vi "Create Indicator in Result.vi"(0 "Result Cluster":refnum<vi>, 1 "Output Clusters in":string[](array[string]), 5 "VI Reference":refnum<vi>, 7 "Ctl Refnum":refnum<vi>, 11 "error in (no error)":errorcluster) -> (4 "Output Clusters out":string[](array[string]), 15 "error out":errorcluster)   [LabVIEW 2021, in "Migrator.lvlib"]
uses:
  Migrator.lvlib
  <vilib>/Utility/miscctls.llb/LVPositionTypeDef.ctl
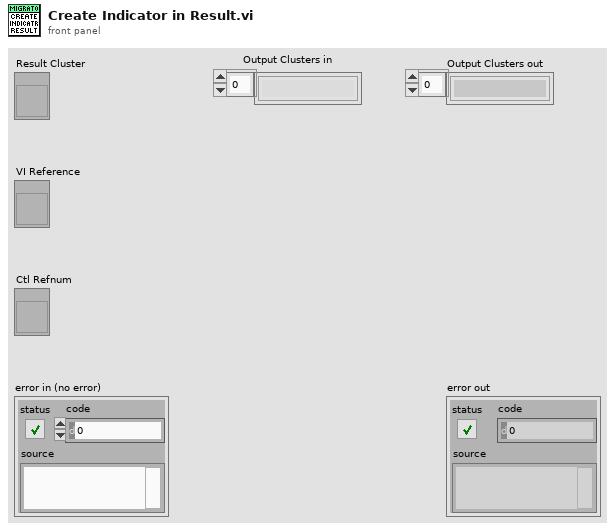
[diagram p1: front panel]
types:
  T1 = typedef "LVPositionTypeDef.ctl" = cluster{"Left":i32, "Top":i32}
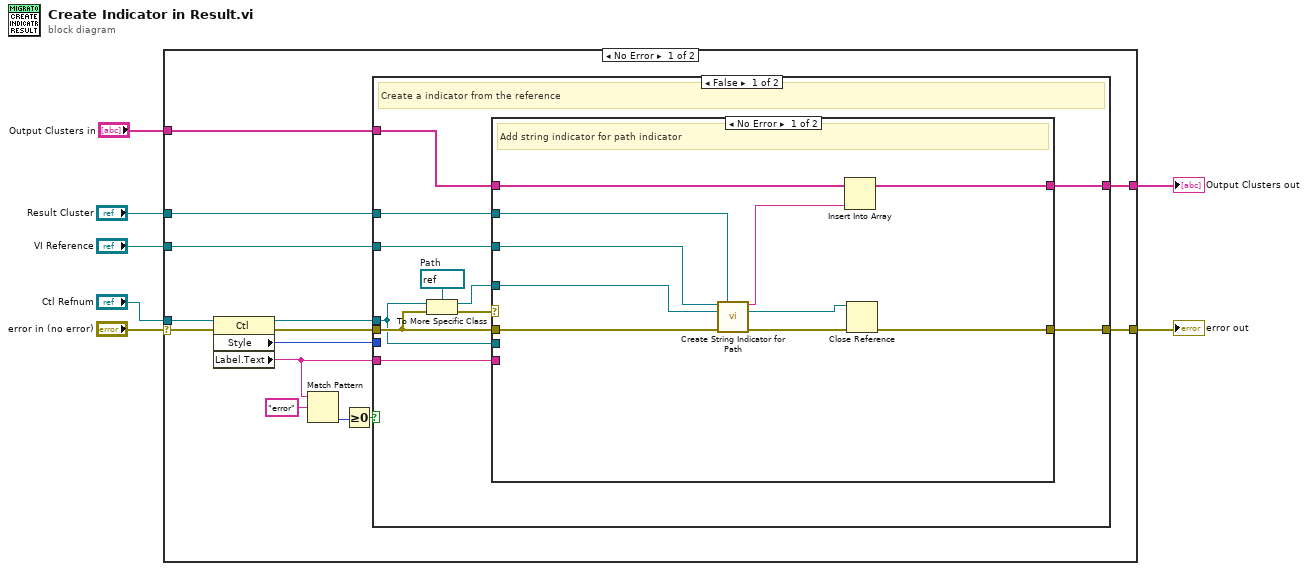
[diagram p0: block diagram]
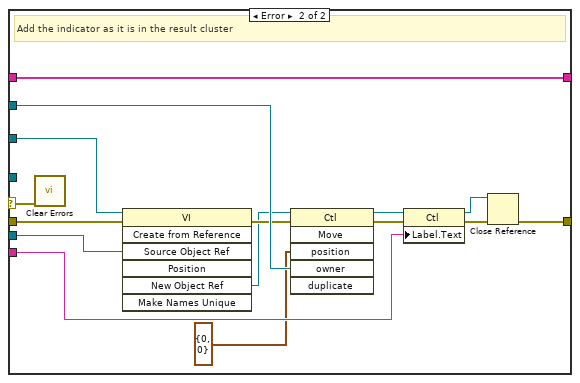
[diagram p2: hidden frame]
diagram:
  n1 = case shown="No Error" "error in (no error)" {
    selector: "error in (no error)" -> [w21 w61]
    tunnel: "Ctl Refnum" -> [w20 _]
    tunnel: "VI Reference" -> [w18 _]
    tunnel: [w13 w61] -> w4
    tunnel: "Result Cluster" -> [w11 _]
    tunnel: "Output Clusters in" -> [w9 w60]
    tunnel: [w8 w60] -> w1
    frame No Error {
      n2 = property class="Ctl"(reference=w20, error in=w21) -> (reference out=w19:refnum<vi>, error out=w12:errorcluster, "Style"=w10:u32, "Label.Text"=w14:string)
      n3 = Match Pattern(string=w14, regular expression="error") -> (offset past match=w16:i32)  [unwired: 1 in, 3 out]
      n4 = Greater Or Equal To 0?(x=w16) -> (x >= 0?=w17:bool)
      n5 = case shown="False" w17 {
        tunnel: w10 -> [_ _]
        tunnel: w11 -> [w30 _]
        tunnel: w12 -> [w27 w59]
        tunnel: w19 -> [w26 _]
        tunnel: [w32 w59] -> w13
        tunnel: w14 -> [w31 _]
        tunnel: w18 -> [w29 _]
        tunnel: w9 -> [w23 w58]
        tunnel: [w22 w58] -> w8
        frame False {
          w28 = refnum<vi> refnum  # Path
          # "Create a indicator from the reference"
          n6 = To More Specific Class(target class=w28, reference=w26, error in=w27) -> (specific class reference=w24:refnum<vi>, error out=w25:errorcluster)
          n7 = case shown="No Error" w25 {
            selector: w25 -> [_ w44]
            tunnel: w27 -> [w42 w57]
            tunnel: [w37 w56] -> w32
            tunnel: w31 -> [_ w55]
            tunnel: w30 -> [w39 w54]
            tunnel: w26 -> [_ w53]
            tunnel: w29 -> [w41 w52]
            tunnel: w24 -> [w40 _]
            tunnel: w23 -> [w34 w43]
            tunnel: [w33 w43] -> w22
            frame No Error {
              # "Add string indicator for path indicator"
              n8 = call "Create String Indicator for Path.vi"("VI Refnum"=w41, "Typedef Cluster"=w39, "Path Refnum"=w40, "error in (no error)"=w42) -> ("Reference String"=w35:string, "String ctl ref"=w36:refnum<vi>, "error out"=w38:errorcluster)  [unwired: 9 in]
              n9 = Insert Into Array(array=w34, new element=w35) -> (w33:string[])  [unwired: 1 in]
              n10 = Close Reference(reference=w36, error in (no error)=w38) -> (error out=w37:errorcluster)
            }
            frame Error {
              # "Add the indicator as it is in the result cluster"
              n11 = call <vilib>:"Clear Errors.vi"("error in (no error)"=w44) -> ()  [unwired: 5 in, 2 out]
              n12 = invoke class="VI" method="Create from Reference"(reference=w52, error in=w57, "Source Object Ref"=w53) -> (error out=w51:errorcluster, "New Object Ref"=w50:refnum<vi>)  [unwired: 4 in, 5 out]
              n13 = invoke class="Ctl" method="Move"(reference=w50, error in=w51, "position"=T1 {"Left"=0, "Top"=0}, "owner"=w54) -> (reference out=w46:refnum<vi>, error out=w48:errorcluster)  [unwired: 2 in, 4 out]
              n14 = property class="Ctl"(reference=w46, error in=w48, "Label.Text"=w55) -> (reference out=w45:refnum<vi>, error out=w47:errorcluster)
              n15 = Close Reference(reference=w45, error in (no error)=w47) -> (error out=w56:errorcluster)
            }
          }
        }
        frame True {
          # "Ignore it is error indicator"
        }
      }
    }
    frame Error {
    }
  }
  "error out" <- w4
  "Output Clusters out" <- w1
